vi "csv temp path.vi"(8 "error in (no error)":errorcluster, 10 "Path_Name":T2, 11 "tdms temp path":path) -> (0 "error out":errorcluster, 2 "A New Folder temp":string, 3 "Table tmp cluster":T1)   [LabVIEW 2018]
panel:
  out "T_Table_tmp_path":path
  out "R_Table_tmp_path":path
  out "S_Table_tmp_path":path
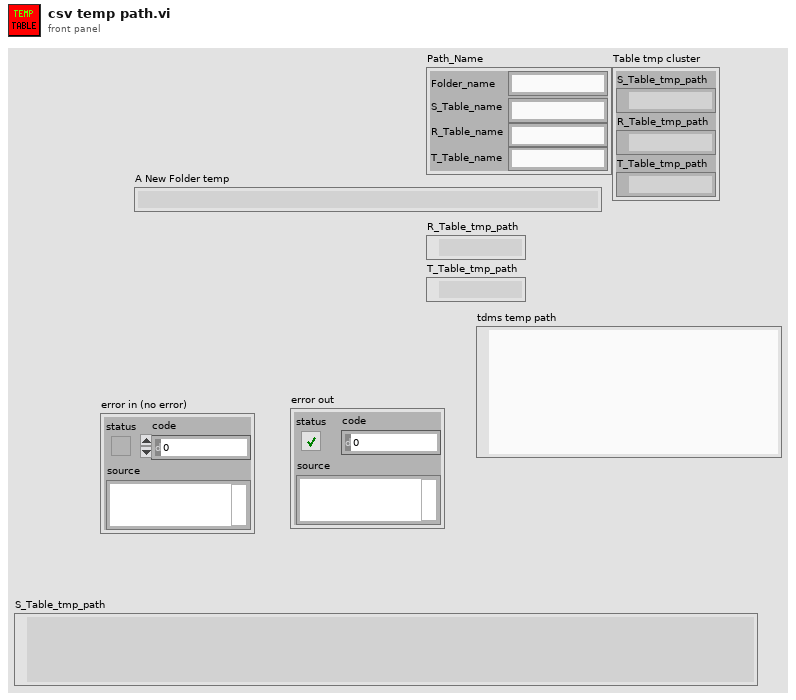
[diagram p1: front panel]
types:
  T1 = cluster{"S_Table_tmp_path":path, "R_Table_tmp_path":path, "T_Table_tmp_path":path}
  T2 = cluster{"Folder_name":string, "S_Table_name":string, "R_Table_name":string, "T_Table_name":string}
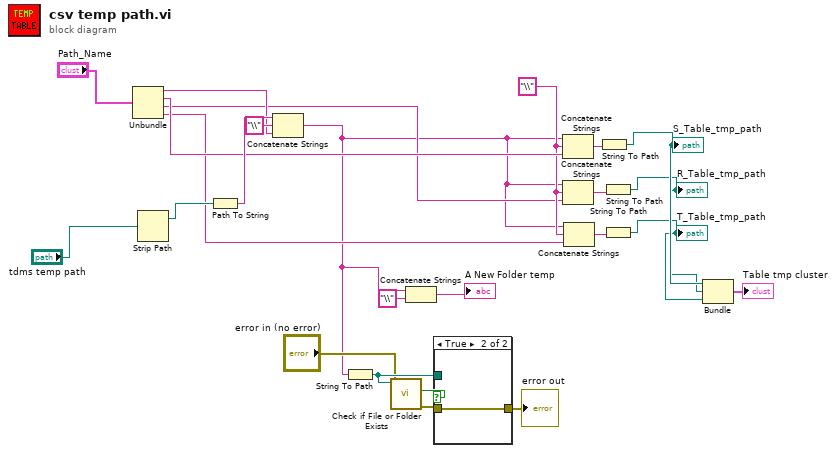
[diagram p0: block diagram]
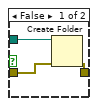
[diagram p2: hidden frame]
diagram:
  w12 = "\\" ("string")
  n1 = Unbundle("Path_Name") -> ("Folder_name"=w15:string, "S_Table_name"=w14:string, "R_Table_name"=w11:string, "T_Table_name"=w10:string)
  n2 = Strip Path(path="tdms temp path") -> (stripped path=w18:path)  [unwired: 1 out]
  n3 = Path To String(path=w18) -> (string=w17:string)
  n4 = Concatenate Strings(w17, "\\" ("string"), w15) -> (w3:string)
  n5 = String To Path(string=w3) -> (path=w25:path)
  n6 = call <vilib>:"Check if File or Folder Exists.vi"("error in (no error)"="error in (no error)", "path"=w25) -> ("error out"=w23:errorcluster, "file or folder exists?"=w24:bool)  [unwired: 7 in, 1 out]
  n7 = Concatenate Strings(w3, "\\" ("string")) -> (→"A New Folder temp":string)
  n8 = case shown="True" w24 {
    tunnel: w25 -> [w28 _]
    tunnel: w23 -> [w27 w29]
    tunnel: [w26 w29] -> w21
    frame False {
      n9 = Create Folder(path (use dialog)=w28, error in=w27) -> (error out=w26:errorcluster)  [unwired: 1 in, 2 out]
    }
    frame True {
    }
  }
  "error out" <- w21
  n10 = Concatenate Strings(w3, w12, w14) -> (w13:string)
  n11 = Concatenate Strings(w3, w12, w11) -> (w9:string)
  n12 = Concatenate Strings(w3, w12, w10) -> (w8:string)
  n13 = String To Path(string=w13) -> (path=w6:path)
  "S_Table_tmp_path" <- w6
  n14 = String To Path(string=w9) -> (path=w5:path)
  "R_Table_tmp_path" <- w5
  n15 = String To Path(string=w8) -> (path=w4:path)
  "T_Table_tmp_path" <- w4
  n16 = Bundle(w6, w5, w4) -> (→"Table tmp cluster":cluster{path, path, path})  [unwired: 1 in]
